vi "DAQmx.Create AO Tasks.vi"(8 "error in (no error)":errorcluster, 11 "DAQmx in":refnum<class "DAQmx.lvclass">) -> (0 "error out":errorcluster, 3 "DAQmx out":refnum<class "DAQmx.lvclass">)   [LabVIEW 2019, in "DAQmx.lvclass"]
uses:
  DAQmx.lvclass
  typedefs/DAQ.Config.AO--Cluster--Array.ctl
  typedefs/DAQ.Config.AO--Cluster.ctl
  typedefs/DAQ.Config.AO.Range--enum.ctl
  typedefs/DAQ.Config.Device Type--enum.ctl
  DAQmx.lvclass/DAQmx.ctl
  <vilib>/DAQmx/create/channels.llb/DAQmx Create Channel (AO-Voltage-Basic).vi
  <resource>/objmgr/daqmx.rc
panel:
  out "AO":T1 {"output terminal configuration" items=[""=-1, "Differential"=10106, "Pseudodifferential"=12529]}
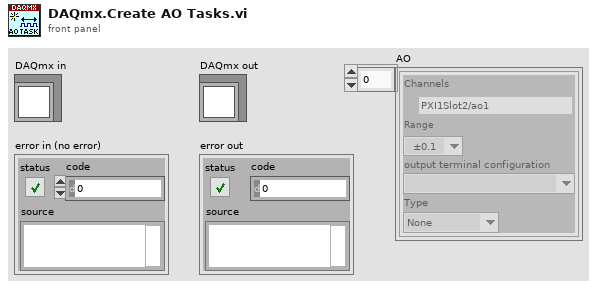
[diagram p1: front panel]
types:
  T1 = typedef "DAQmx.lvclass/DAQ.Config.AO--Cluster--Array.ctl" = T2[]
  T2 = typedef "DAQmx.lvclass/DAQ.Config.AO--Cluster.ctl" = cluster{"Channels":tag, "Range":T3, "output terminal configuration":i32, "Type":T4}
  T3 = typedef "DAQmx.lvclass/DAQ.Config.AO.Range--enum.ctl" = enum16{"±0.1", "±1.0", "±3.5", "±10.0", ""}
  T4 = typedef "DAQmx.lvclass/DAQ.Config.Device Type--enum.ctl" = enum16{"None", "USB-4431", "PXI-446x"}
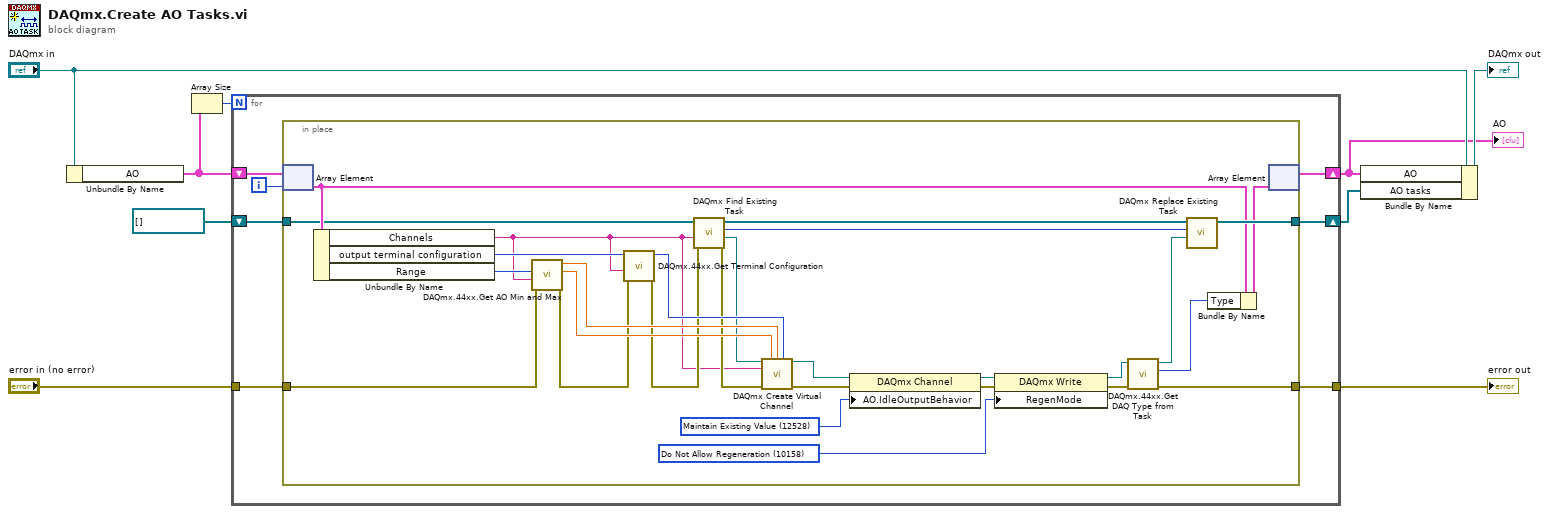
[diagram p0: block diagram]
diagram:
  n1 = Unbundle By Name("DAQmx in") -> ("AO"=w2:T1)
  n2 = Array Size(array=w2) -> (size(s)=w3:i32)
  n3 = for {
    N: w3 -> [_]
    tunnel: "error in (no error)" -> [w16]
    tunnel: [w15] -> w4
    shift-right: [w14] -> w6
    shift-left: refnum<k21>[] [] -> [w13]
    shift-right: [w11] -> w1
    shift-left: w2 -> [w12]
    i -> [w10]
    n4 = in-place {
      in-place-border: w16 -> [w44]
      in-place-border: [w42] -> w15
      in-place-border: [w34] -> w14
      in-place-border: w13 -> [w19]
      w38 = 10158 items=["Allow Regeneration"=10097, "Do Not Allow Regeneration"=10158] ("RegenMode")
      w37 = 12528 items=["Zero Volts"=12526, "High-Impedance"=12527, "Maintain Existing Value"=12528] ("AO.IdleOutputBehavior")
      n5 = in-place-array #1(w12, w10) -> (w22:T2)
      n6 = Unbundle By Name(w22) -> ("Channels"=w18:tag, "output terminal configuration"=w23:i32, "Range"=w21:T3)
      n7 = call "DAQmx.44xx.Get AO Min and Max.vi"("error in (no error)"=w44, "AO.channels"=w18, "AO.Range"=w21) -> ("error out"=w27:errorcluster, "AO.max"=w29:dbl, "AO.min"=w28:dbl)  [unwired: 6 in]
      n8 = call "DAQmx.44xx.Get Terminal Configuration.vi"("error in (no error)"=w27, "Channel in"=w18, "terminal configuration in"=w23) -> ("error out"=w26:errorcluster, "terminal configuration out"=w30:i32)  [unwired: 7 in]
      n9 = call "DAQmx Find Existing Task.vi"("error in (no error)"=w26, "Channels"=w18, "Tasks in"=w19) -> ("error out"=w25:errorcluster, "Task out"=w17:refnum<k21>, "Task Index"=w24:i32, "Tasks out"=w20:refnum<k21>[])  [unwired: 5 in]
      n10 = call-poly <vilib>:"DAQmx Create Virtual Channel.vi"("task in"=w17, "maximum value"=w29, "minimum value"=w28, "output terminal configuration"=w30, "physical channels"=w18, "error in"=w25) -> ("task out"=w36:refnum<k21>, "error out"=w41:errorcluster)  [unwired: 8 in]
      n11 = property class="DAQmx Channel"(reference=w36, error in=w41, "AO.IdleOutputBehavior"=w37) -> (reference out=w40:refnum<k21>, error out=w39:errorcluster)
      n12 = property class="DAQmx Write"(reference=w40, error in=w39, "RegenMode"=w38) -> (reference out=w35:refnum<k21>, error out=w43:errorcluster)
      n13 = call "DAQmx.44xx.Get DAQ Type from Task.vi"("error in (no error)"=w43, "Task in"=w35) -> ("error out"=w42:errorcluster, "DAQ Type"=w32:T4, "Task out"=w33:refnum<k21>)  [unwired: 5 in, 2 out]
      n14 = call "DAQmx Replace Existing Task.vi"("Task in"=w33, "Task Index"=w24, "Tasks in"=w20) -> ("Tasks out"=w34:refnum<k21>[])  [unwired: 8 in]
      n15 = Bundle By Name(cluster=w22, "Type"=w32) -> (w31:T2)
      n16 = in-place-array #1(w31) -> (w11:T1)  [unwired: 1 out]
    }
  }
  "error out" <- w4
  "AO" <- w1
  n17 = Bundle By Name(cluster="DAQmx in", "AO"=w1, "AO tasks"=w6) -> (→"DAQmx out":refnum<class "DAQmx.lvclass">)
